vi "VM - Context Names.vi"(6 "error in":errorcluster, 7 "action":T1(ring), 8 "VC Name":string, 9 "VC Handle":T2=-1) -> (0 "error out":errorcluster, 1 "error code":u16(ring) items=["no error", "wrong name", "name not found", "non-unique name", "invalid handle", "unknown error"], 2 "VC Name out":string, 3 "VC Handle out":T2=-1)   [LabVIEW 2021]
doc: "This VI manages the names of local contexts. Every context can have a unique name that consists of any printable characters (a name cannot start with blanks). Refer to the VI help for more details.\n\n<b>VC Handle</b> control specifies the handle of a variable context.\n\n<b>VC Name</b> control specifies the name of the context. It is used to assign a name to the context and to retrieve the context handle through its name.\n\n<b>action</b> control specifies the operation to perform:\n 'nothing' : does nothing.\n 'reset' : clears all assigned name entries.\n 'assign name' : assigns a name to the given context (<b>VC Handle</b>).\n 'get name' : returns the name assigned to the given context (<b>VC Handle</b>).\n 'get handle' : returns the handle of the context that has the given <b>VC Name</b>.\n\n<b>VC Name out</b> indicator returns the name of the given context.\n\n::: CalcExpress Toolkit :::\nCopyright (c) 2000-2026 Konstantin Shifershteyn. All rights reserved."
uses:
  cetypes.llb/VarMan Variable Context Handle.ctl
  cetypes.llb/VarMan Error Code.ctl
  cersrc/celveng32.dll
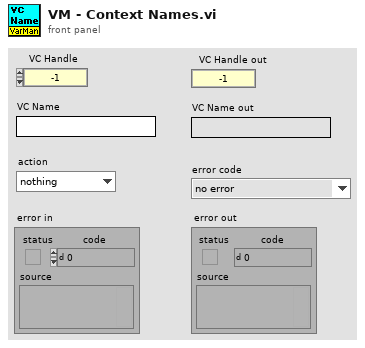
[diagram p1: front panel]
types:
  T1 = enum32{"nothing", "reset", "assign name", "get name", "get handle"}
  T2 = typedef "VarMan Variable Context Handle.ctl" = i32
  T3 = typedef "VarMan Error Code.ctl" = u16
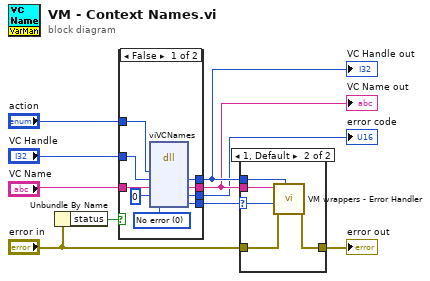
[diagram p0: block diagram]
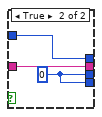
[diagram p2: hidden frame]
diagram:
  n1 = Unbundle By Name("error in") -> ("status"=w8:bool)
  n2 = case shown="False" w8 {
    tunnel: "VC Handle" -> [w13 w21]
    tunnel: "VC Name" -> [w14 w22]
    tunnel: [w17 w20] -> w2
    tunnel: [w19 w21] -> w5
    tunnel: [w18 w22] -> w4
    tunnel: "action" -> [w12 _]
    tunnel: [w16 w20] -> w1
    frame False {
      w11 = T3 0 items=["No error", "Invalid variable type", "Variable not found", "Variable already exists", "Invalid context handle", "Input error", "Invalid data format", "No history attached", "History already attached", "Invalid history parameters", "Wrong variable name", "Wrong alias name", "Non-unique alias", "Alias not found", "No alias associated", "Alias already associated", "Wrong context name", "Non-unique context name", "Context name not found", "Invalid parameter", "Generic error", "Memory Full", "Unrecognized LV error", "Unknown error code"] ("VarMan error")
      n3 = dll-call lib="C:/LV Projects/CalcExpress 40 LV2021/vi.lib/addons/CalcExpress/cersrc/celveng*.dll" fn="viVCNames"("cmd"=w12, "vch"=w13, "vcName"=w14, "viErrc"=u16 0, "vmErrc"=w11) -> ("vch"=w19:T2, "vcName"=w18:string, "viErrc"=w17:u16, "vmErrc"=w16:T3)  [unwired: 5 in, 2 out]
    }
    frame True {
      w20 = u16 0
    }
  }
  "VC Handle out" <- w5
  "VC Name out" <- w4
  "error code" <- w2
  n4 = case shown="1, Default" w1 {
    selector: w1 -> [_ w24]
    tunnel: w4 -> [_ w27]
    tunnel: "error in" -> [w23 w26]
    tunnel: [w23 w25] -> w10
    tunnel: w5 -> [_ w28]
    frame 0 {
    }
    frame 1, Default {
      n5 = call "VM wrappers - Error Handler.vi"("VC Handle"=w28, "error before"=w26, "VarMan error"=w24, "name spec"=w27) -> ("error out"=w25:errorcluster)  [unwired: 6 in, 1 out]
    }
  }
  "error out" <- w10
